vi "VIH ProjFile - Cluster - Read.vi"(8 "error in":errorcluster, 10 "Ctl Refnum":refnum<vi>, 11 "XML Parent Item":refnum<k20>) -> (0 "error out":errorcluster, 3 "dup XML Parent Item":refnum<k20>)   [LabVIEW 2014]
doc: "::: VI Helpeks :::\nCopyright (c) 2000-2026 Konstantin Shifershteyn. All rights reserved."
uses:
  <vilib>/xml/Close Reference(Node).vi
  <resource>/objmgr/DOMUserDefRef.rc
  <vilib>/xml/NI_XML.lvlib
panel:
  # "VI Helpeks\nCopyright (c) 2012-2026 Konstantin Shifershteyn"
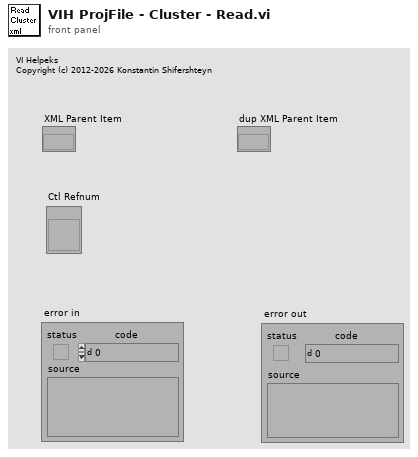
[diagram p1: front panel]
types:
  T1 = typedef "LVStringsAndValuesArrayTypeDef.ctl" = cluster{"String":string, "Value":ext}[]
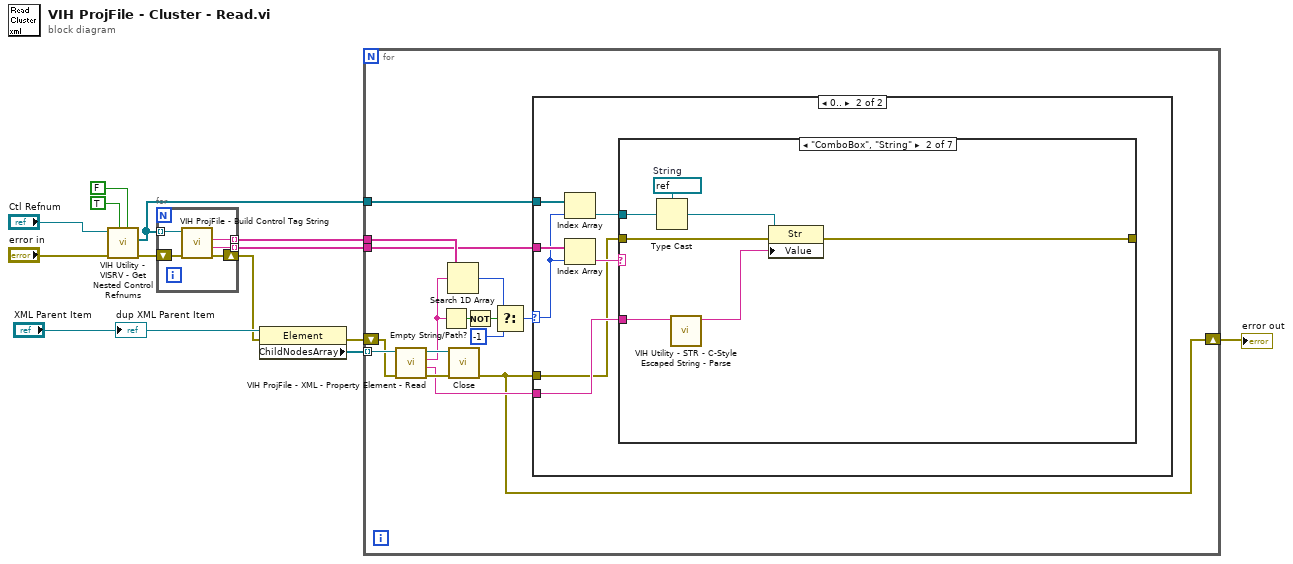
[diagram p0: block diagram]
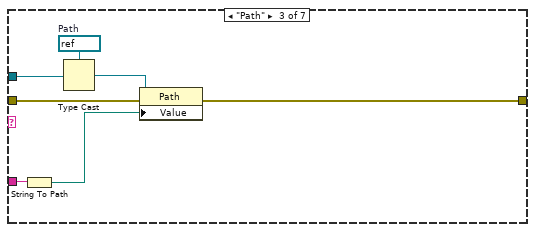
[diagram p4: hidden frame]
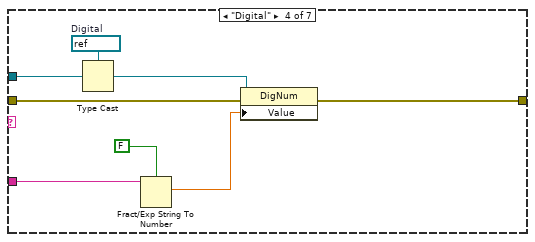
[diagram p5: hidden frame]
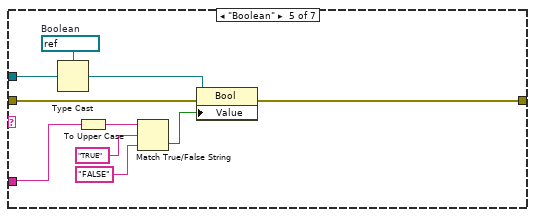
[diagram p6: hidden frame]
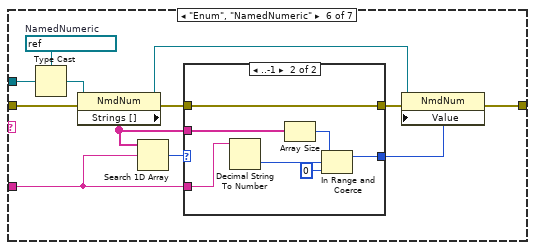
[diagram p7: hidden frame]
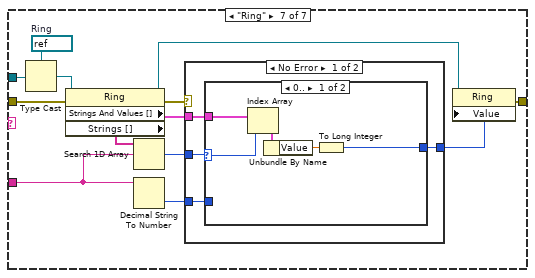
[diagram p9: hidden frame]
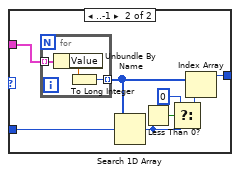
[diagram p10: hidden frame]
diagram:
  n1 = call "VIH Utility - VISRV - Get Nested Control Refnums.vi"("array element (T)"=FALSE, "cluster members (T)"=TRUE, "error in"="error in", "Ctl Refnum"="Ctl Refnum") -> ("error out"=w10:errorcluster, "nested Ctl Refnums"=w3:refnum<vi>[])  [unwired: 5 in, 1 out]
  n2 = for {
    tunnel: w3 -> [w18] mode=indexing
    shift-right: [w16] -> w5
    shift-left: w10 -> [w17]
    tunnel: [w14] -> w4 mode=indexing
    tunnel: [w15] -> w2 mode=indexing
    n3 = call "VIH ProjFile - Build Control Tag String.vi"("error in"=w17, "Ctl Refnum"=w18) -> ("error out"=w16:errorcluster, "Control Class"=w15:string, "Control Tag"=w14:string)  [unwired: 5 in, 2 out]
  }
  n4 = property class="Element"(reference="XML Parent Item", error in=w5) -> (error out=w8:errorcluster, "ChildNodesArray"=w7:refnum<k20>[])  [unwired: 1 out]
  n5 = for {
    shift-right: [w19] -> w1
    shift-left: w8 -> [w30]
    tunnel: w7 -> [w33] mode=indexing
    tunnel: w4 -> [w29]
    tunnel: w3 -> [w22]
    tunnel: w2 -> [w21]
    n6 = call "VIH ProjFile - XML - Property Element - Read.vi"("error in"=w30, "XML Node"=w33) -> ("error out"=w31:errorcluster, "Property Value"=w20:string, "Property Name"=w28:string, "dup XML Node"=w32:refnum<k20>)  [unwired: 6 in]
    n7 = Empty String/Path?(string/path=w28) -> (empty?=w27:bool)
    n8 = Search 1D Array(1D array=w29, element=w28) -> (index of element=w25:i32)  [unwired: 1 in]
    n9 = call-poly <vilib>:"Close.vi"("error in (no error)"=w31, "node"=w32) -> ("error out"=w19:errorcluster)  [unwired: 7 in]
    n10 = Not(x=w27) -> (.not. x?=w26:bool)
    n11 = Select(t=w25, s=w26, f=-1) -> (s? t:f=w23:i32)
    n12 = case shown="0.." w23 {
      selector: w23 -> [_ w38]
      tunnel: w22 -> [_ w40]
      tunnel: w21 -> [_ w39]
      tunnel: w20 -> [_ w35]
      tunnel: w19 -> [_ w34]
      frame ..-1 {
      }
      frame 0.. {
        n13 = Index Array(array=w40, index=w38) -> (element=w36:refnum<vi>)
        n14 = Index Array(array=w39, index=w38) -> (element=w37:string)
        n15 = case shown="\"ComboBox\", \"String\"" w37 {
          tunnel: w36 -> [_ w47 w52 w59 w67 w76 w97]
          tunnel: w34 -> [w41 w46 w49 w56 w68 w77 w98]
          tunnel: [w41 w48 w55 w63 w69 w82 w106] -> _
          tunnel: w35 -> [_ w43 w54 w61 w70 w79 w101]
          frame Default {
          }
          frame "ComboBox", "String" {
            w45 = refnum<vi> refnum  # String
            n16 = Type Cast(type=w45, x=w47) -> (*(type *) &x=w44:refnum<vi>)
            n17 = call "VIH Utility - STR - C-Style Escaped String - Parse.vi"("String in"=w43) -> ("String out"=w42:string)  [unwired: 10 in]
            n18 = property class="Str"(reference=w44, error in=w46, "Value"=w42) -> (error out=w48:errorcluster)  [unwired: 1 out]
          }
          frame "Path" {
            w51 = refnum<vi> refnum  # Path
            n19 = String To Path(string=w54) -> (path=w53:path)
            n20 = Type Cast(type=w51, x=w52) -> (*(type *) &x=w50:refnum<vi>)
            n21 = property class="Path"(reference=w50, error in=w49, "Value"=w53) -> (error out=w55:errorcluster)  [unwired: 1 out]
          }
          frame "Digital" {
            w58 = refnum<vi> refnum  # Digital
            n22 = Type Cast(type=w58, x=w59) -> (*(type *) &x=w57:refnum<vi>)
            n23 = Fract/Exp String To Number(use system decimal point (T)=FALSE ("system decimal point (F)"), string=w61) -> (number=w62:dbl)  [unwired: 3 out]
            n24 = property class="DigNum"(reference=w57, error in=w56, "Value"=w62) -> (error out=w63:errorcluster)  [unwired: 1 out]
          }
          frame "Boolean" {
            w66 = refnum<vi> refnum  # Boolean
            n25 = Type Cast(type=w66, x=w67) -> (*(type *) &x=w65:refnum<vi>)
            n26 = To Upper Case(1:w70) -> (0:w64:string)
            n27 = Match True/False String(2:"FALSE" ("false string"), 3:"TRUE" ("true string"), 4:w64) -> (0:w73:bool)  [unwired: 1 out]
            n28 = property class="Bool"(reference=w65, error in=w68, "Value"=w73) -> (error out=w69:errorcluster)  [unwired: 1 out]
          }
          frame "Enum", "NamedNumeric" {
            w75 = refnum<vi> refnum  # NamedNumeric
            n29 = Type Cast(type=w75, x=w76) -> (*(type *) &x=w74:refnum<vi>)
            n30 = property class="NmdNum"(reference=w74, error in=w77) -> (reference out=w81:refnum<vi>, error out=w85:errorcluster, "Strings []"=w78:string[])
            n31 = Search 1D Array(1D array=w78, element=w79) -> (index of element=w84:i32)  [unwired: 1 out]
            n32 = case shown="..-1" w84 {
              selector: w84 -> [w86 _]
              tunnel: w85 -> [w87 w94]
              tunnel: [w87 w94] -> w83
              tunnel: [w86 w92] -> w80
              tunnel: w79 -> [_ w93]
              tunnel: w78 -> [_ w88]
              frame 0.. {
              }
              frame ..-1 {
                n33 = Decimal String To Number(string=w93) -> (number=w91:i32)  [unwired: 3 out]
                n34 = Array Size(array=w88) -> (size(s)=w89:i32)
                n35 = In Range and Coerce(upper limit=w89, x=w91, lower limit=0) -> (coerced(x)=w92:i32)  [unwired: 1 out]
              }
            }
            n36 = property class="NmdNum"(reference=w81, error in=w83, "Value"=w80) -> (error out=w82:errorcluster)  [unwired: 1 out]
          }
          frame "Ring" {
            w95 = refnum<vi> refnum  # Ring
            n37 = Type Cast(type=w95, x=w97) -> (*(type *) &x=w96:refnum<vi>)
            n38 = property class="Ring"(reference=w96, error in=w98) -> (reference out=w105:refnum<vi>, error out=w99:errorcluster, "Strings And Values []"=w102:T1, "Strings []"=w103:string[])
            n39 = Search 1D Array(1D array=w103, element=w101) -> (index of element=w107:i32)  [unwired: 1 out]
            n40 = Decimal String To Number(string=w101) -> (number=w100:i32)  [unwired: 3 out]
            n41 = case shown="No Error" w99 {
              tunnel: w107 -> [w111 _]
              tunnel: [w110 w128] -> w104
              tunnel: w102 -> [w109 _]
              tunnel: w100 -> [w108 w128]
              frame No Error {
                n42 = case shown="0.." w111 {
                  selector: w111 -> [w115 _]
                  tunnel: [w112 w124] -> w110
                  tunnel: w109 -> [w116 w123]
                  tunnel: w108 -> [_ w122]
                  frame 0.. {
                    n43 = Index Array(array=w116, index=w115) -> (element=w114:cluster{"String":string, "Value":ext})
                    n44 = Unbundle By Name(w114) -> ("Value"=w113:ext)
                    n45 = To Long Integer(number=w113) -> (32bit integer=w112:i32)
                  }
                  frame ..-1 {
                    n46 = for {
                      tunnel: w123 -> [w127] mode=indexing
                      tunnel: [w125] -> w121 mode=indexing
                      n47 = Unbundle By Name(w127) -> ("Value"=w126:ext)
                      n48 = To Long Integer(number=w126) -> (32bit integer=w125:i32)
                    }
                    n49 = Search 1D Array(1D array=w121, element=w122) -> (index of element=w120:i32)  [unwired: 1 out]
                    n50 = Less Than 0?(x=w120) -> (x < 0?=w119:bool)
                    n51 = Select(t=0, s=w119, f=w120) -> (s? t:f=w118:i32)
                    n52 = Index Array(array=w121, index=w118) -> (element=w124:i32)
                  }
                }
              }
              frame Error {
              }
            }
            n53 = property class="Ring"(reference=w105, "Value"=w104) -> (error out=w106:errorcluster)  [unwired: 1 in, 1 out]
          }
        }
      }
    }
  }
  "error out" <- w1
  "dup XML Parent Item" <- "XML Parent Item"
